vi "user32 GetSysColor.vi"(0 "nIndex":i32=13, 11 "error in":errorcluster) -> (4 "color":u32, 15 "error out":errorcluster)   [LabVIEW 2020, in "RemoteVI.lvlib"]
doc: "Returns the colour of a Windows display element through user32.dll GetSysColor (stdcall, called in any thread), as a COLORREF 0x00BBGGRR (red in the low byte). nIndex 13 COLOR_HIGHLIGHT is the background of a selected menu item. When error in carries an error the DLL is not called. Generated by scripts\\Build Win32 Wrappers.vi - do not edit by hand, rebuild it."
uses:
  RemoteVI.lvlib
  user32.dll
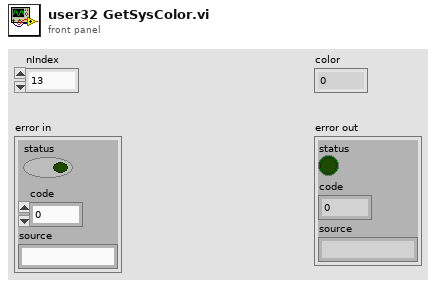
[diagram p1: front panel]
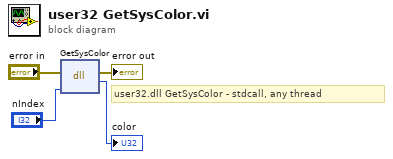
[diagram p0: block diagram]
diagram:
  # "user32.dll GetSysColor - stdcall, any thread"
  n1 = dll-call lib="user32.dll" fn="GetSysColor"(error in="error in", "nIndex"="nIndex") -> (error out=→"error out":errorcluster, →"color":u32)  [unwired: 3 in, 1 out]
